vi "FuncVI_Sub - Script - Save Script Paths.vi"(7 "Caller CSE RefNum":T1, 8 "error in":errorcluster, 10 "Script File Path":path, 11 "CSE RefNum":T1) -> (0 "error out":errorcluster, 3 "dup CSE RefNum":T1)   [LabVIEW 2021]
doc: "::: CalcExpress Toolkit :::\nCopyright (c) 2000-2026 Konstantin Shifershteyn. All rights reserved."
uses:
  cse.llb/CSE Instance RefNum.ctl
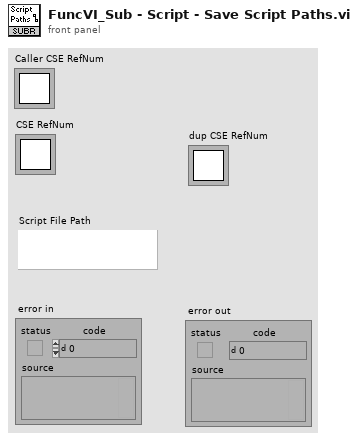
[diagram p1: front panel]
types:
  T1 = typedef "CSE Instance RefNum.ctl" = refnum<k1>
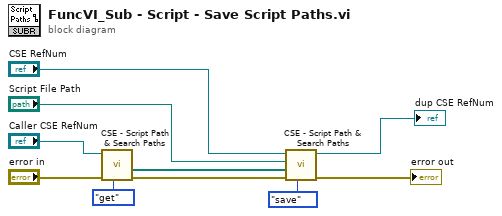
[diagram p0: block diagram]
diagram:
  n1 = call "CSE - Script Path & Search Paths.vi"("action"=enum32{"get", "save"}."get", "error in"="error in", "CSE RefNum"="Caller CSE RefNum") -> ("error out"=w8:errorcluster, "search paths out"=w6:path[])  [unwired: 5 in, 2 out]
  n2 = call "CSE - Script Path & Search Paths.vi"("action"=enum32{"get", "save"}."save", "error in"=w8, "search paths"=w6, "script file path"="Script File Path", "CSE RefNum"="CSE RefNum") -> ("error out"=→"error out":errorcluster, "dup CSE RefNum"=→"dup CSE RefNum":T1)  [unwired: 3 in, 2 out]
